vi "Self Alignment.vi"(8 "error in (no error)":errorcluster caption="에러 입력(에러 없음)", 11 "Instrument Manager 입력":refnum<class "Instrument Manager.lvclass">) -> (0 "error out":errorcluster caption="에러 출력", 3 "Instrument Manager 출력":refnum<class "Instrument Manager.lvclass">)   [LabVIEW 2023, in "Instrument Manager.lvclass"]
uses:
  Instrument Manager.lvclass
  Instrument Manager.lvclass/Instrument Manager.ctl
  Module/Spectrum Analyzer/Interface_Spectrum/Interface_Spectrum.lvclass
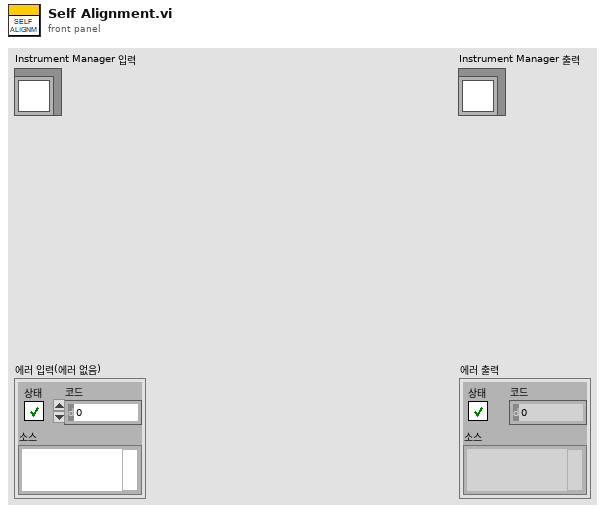
[diagram p1: front panel]
types:
  T1 = cluster{"Anritsu Call Box":refnum<class "Anritsu Call Box.lvclass">, "Spectrum Analyzer":refnum<class "Interface_Spectrum.lvclass">, "RF Switch Box":refnum<class "RF Filter Box.lvclass">, "Turn Table":refnum<class "Interface - Turn Table.lvclass">, "Mast":refnum<class "Interface - Mast.lvclass">, "3D Controller":refnum<class "Interface_3D Controller.lvclass">}
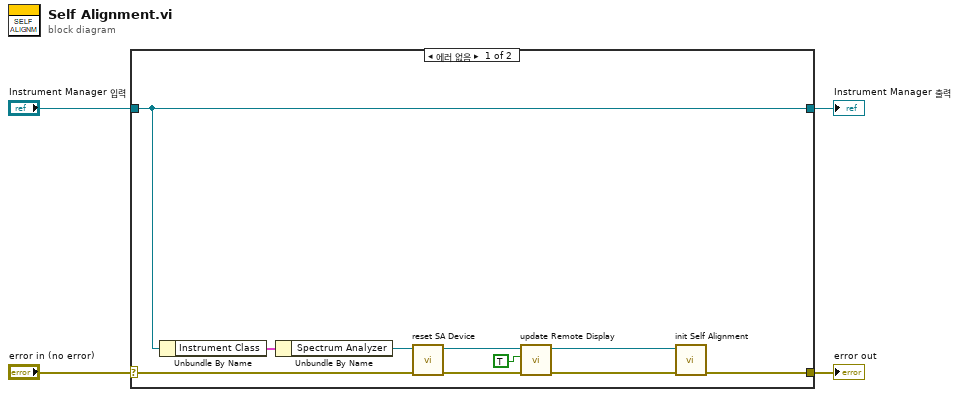
[diagram p0: block diagram]
diagram:
  n1 = case shown="에러 없음" "error in (no error)" {
    selector: "error in (no error)" -> [w14 w16]
    tunnel: [w13 w16] -> w3
    tunnel: [w12 w15] -> w1
    tunnel: "Instrument Manager 입력" -> [w12 w15]
    frame No Error {
      n2 = Unbundle By Name(w12) -> ("Instrument Class"=w11:T1)
      n3 = Unbundle By Name(w11) -> ("Spectrum Analyzer"=w10:refnum<class "Interface_Spectrum.lvclass">)
      n4 = call-dynamic "reset SA Device.vi"("error in (no error)"=w14, "Interface_Spectrum in"=w10) -> ("error out"=w8:errorcluster, "Interface_Spectrum out"=w9:refnum<class "Interface_Spectrum.lvclass">)  [unwired: 8 in]
      n5 = call-dynamic "update Remote Display.vi"("error in (no error)"=w8, "Remote Display On?"=TRUE, "Interface_Spectrum in"=w9) -> ("error out"=w7:errorcluster, "Interface_Spectrum out"=w6:refnum<class "Interface_Spectrum.lvclass">)  [unwired: 7 in]
      n6 = call-dynamic "init Self Alignment.vi"("error in (no error)"=w7, "Interface_Spectrum in"=w6) -> ("error out"=w13:errorcluster)  [unwired: 8 in, 1 out]
    }
    frame Error {
    }
  }
  "error out" <- w3
  "Instrument Manager 출력" <- w1
